vi "Lab9_RT.vi"() -> ()   [LabVIEW 2025]
panel:
  out "usage %":dbl
  out "CPU [%]":dbl
  out "error out":errorcluster
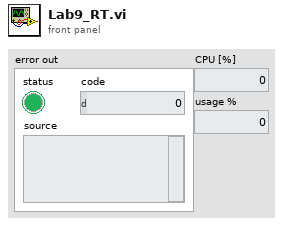
[diagram p1: front panel]
types:
  T1 = typedef "Logger_State.ctl" = cluster{"ref TDMS":refnum<k34>, "File Path":path, "counter":i32, "Folder tmp":path, "folder ready":path}
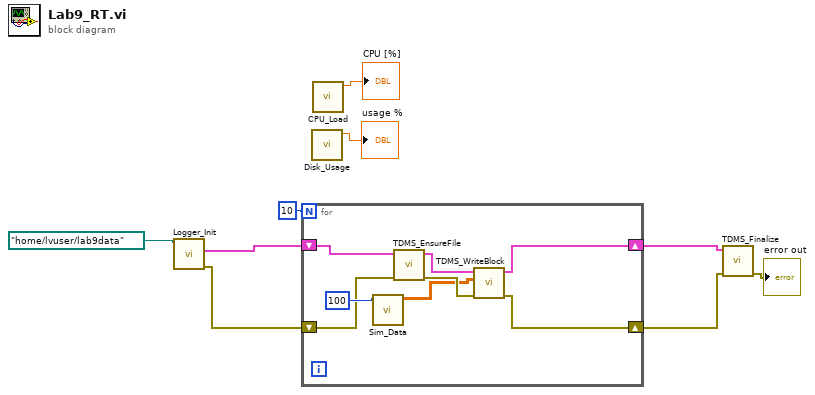
[diagram p0: block diagram]
diagram:
  n1 = call "Logger_Init.vi"("base path"=path "/home/lvuser/lab9data") -> ("error out"=w7:errorcluster, "state"=w6:T1)  [unwired: 8 in, 1 out]
  n2 = for {
    N: 10 -> [_]
    shift-right: [w10] -> w5
    shift-left: w6 -> [w16]
    shift-right: [w13] -> w4
    shift-left: w7 -> [w15]
    n3 = call "Sim_Data.vi"("Number in"=100) -> ("data"=w12:dbl[][])  [unwired: 10 in]
    n4 = call "TDMS_EnsureFile.vi"("error in (no error)"=w15, "Logger_state"=w16) -> ("error out"=w14:errorcluster, "state out"=w11:T1)  [unwired: 8 in]
    n5 = call "TDMS_WriteBlock.vi"("error in (no error)"=w14, "Array"=w12, "Logger_state"=w11) -> ("error out"=w13:errorcluster, "state out"=w10:T1)  [unwired: 7 in]
  }
  n6 = call "Disk_Usage.vi"() -> ("usage %"=→"usage %":dbl)  [unwired: 11 in]
  n7 = call "CPU_Load.vi"() -> ("CPU [%]"=→"CPU [%]":dbl)  [unwired: 11 in]
  n8 = call "TDMS_Finalize.vi"("error in (no error)"=w4, "state in"=w5) -> ("error out"=→"error out":errorcluster)  [unwired: 9 in]
